vi "Post-Uninstall Custom Action.vi"(10 "Variant":variant) -> (0 "error out":errorcluster)   [LabVIEW 2024]
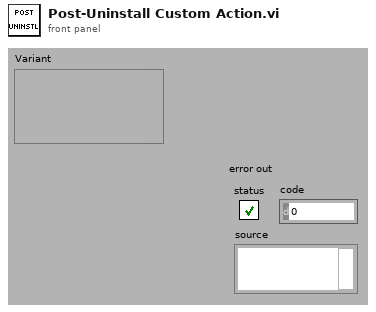
[diagram p1: front panel]
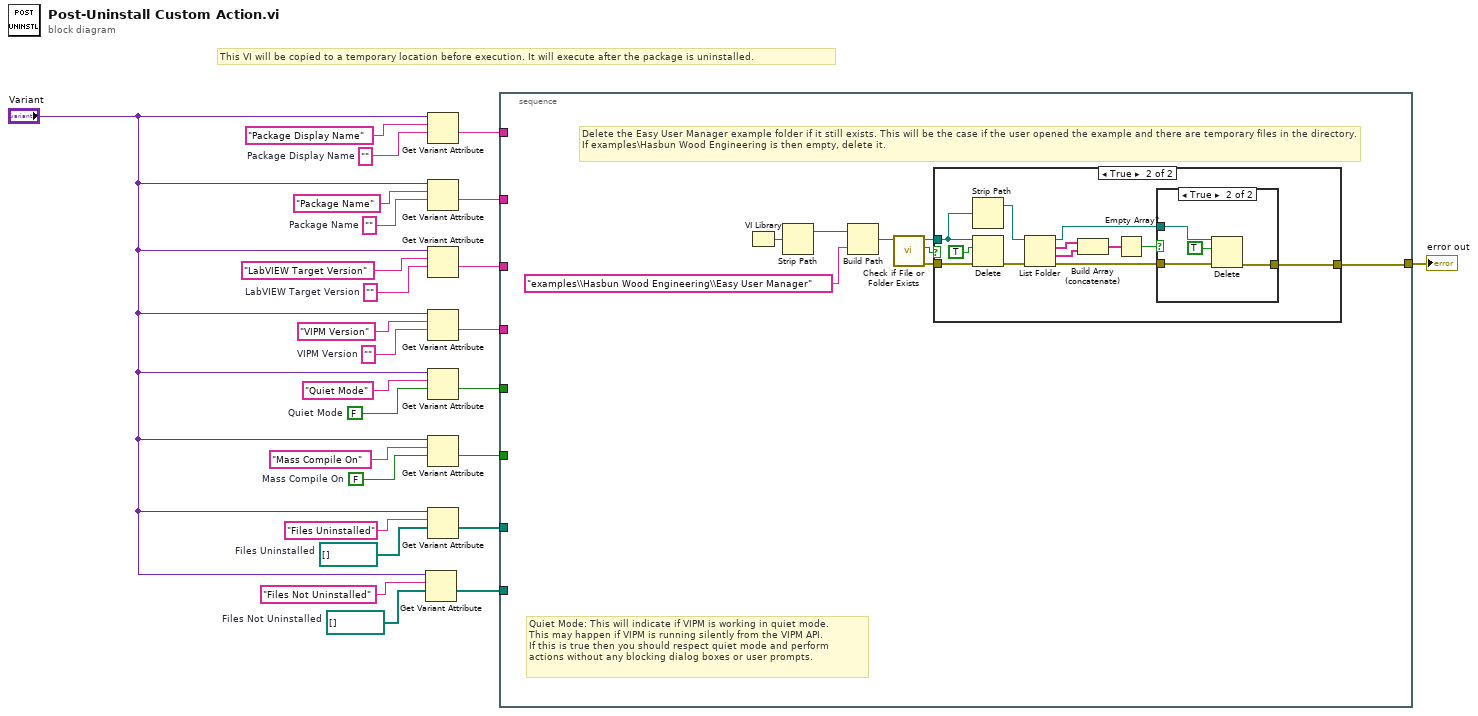
[diagram p0: block diagram]
diagram:
  w2 = path[] []  # Files Not Uninstalled
  w3 = path[] []  # Files Uninstalled
  w9 = FALSE  # Mass Compile On
  w10 = ""  # Package Display Name
  w17 = FALSE  # Quiet Mode
  w20 = ""  # VIPM Version
  w22 = ""  # LabVIEW Target Version
  w24 = ""  # Package Name
  # "This VI will be copied to a temporary location before execution. It will execute after the package is uninstalled."
  n1 = Get Variant Attribute(Variant="Variant", name="Files Not Uninstalled", default value (empty Variant)=w2) -> (value=w7:path[])  [unwired: 1 in, 3 out]
  n2 = Get Variant Attribute(Variant="Variant", name="Package Display Name", default value (empty Variant)=w10) -> (value=w16:string)  [unwired: 1 in, 3 out]
  n3 = Get Variant Attribute(Variant="Variant", name="Package Name", default value (empty Variant)=w24) -> (value=w15:string)  [unwired: 1 in, 3 out]
  n4 = Get Variant Attribute(Variant="Variant", name="LabVIEW Target Version", default value (empty Variant)=w22) -> (value=w14:string)  [unwired: 1 in, 3 out]
  n5 = Get Variant Attribute(Variant="Variant", name="VIPM Version", default value (empty Variant)=w20) -> (value=w13:string)  [unwired: 1 in, 3 out]
  n6 = Get Variant Attribute(Variant="Variant", name="Quiet Mode", default value (empty Variant)=w17) -> (value=w12:bool)  [unwired: 1 in, 3 out]
  n7 = Get Variant Attribute(Variant="Variant", name="Mass Compile On", default value (empty Variant)=w9) -> (value=w11:bool)  [unwired: 1 in, 3 out]
  n8 = Get Variant Attribute(Variant="Variant", name="Files Uninstalled", default value (empty Variant)=w3) -> (value=w6:path[])  [unwired: 1 in, 3 out]
  n9 = stacked-sequence {
    tunnel: w16 -> [_]
    tunnel: w15 -> [_]
    tunnel: w14 -> [_]
    tunnel: w13 -> [_]
    tunnel: w12 -> [_]
    tunnel: w11 -> [_]
    tunnel: w6 -> [_]
    tunnel: w7 -> [_]
    tunnel: [w27] -> w1
    frame #0 {
      # "Quiet Mode: This will indicate if VIPM is working in quiet mode.\nThis may happen if VIPM is running silently from the VIPM API.\nIf this is true then you should respect quiet mode and perform\nactions without any blocking dialog boxes or user prompts."
      # "Delete the Easy User Manager example folder if it still exists. This will be the case if the user opened the example and there are temporary files in the directory. If examples\\Hasbun Wood Engineering is then empty, delete it."
      n10 = VI Library() -> (path=w34:path)
      n11 = Strip Path(path=w34) -> (stripped path=w33:path)  [unwired: 1 out]
      n12 = Build Path(base path=w33, name or relative path="examples\\Hasbun Wood Engineering\\Easy User Manager") -> (appended path=w28:path)
      n13 = call <vilib>:"Check if File or Folder Exists.vi"("path"=w28) -> ("error out"=w29:errorcluster, "file or folder exists?"=w31:bool, "dup path"=w30:path)  [unwired: 8 in]
      n14 = case shown="True" w31 {
        tunnel: w30 -> [_ w36]
        tunnel: w29 -> [w35 w47]
        tunnel: [w35 w37] -> w27
        frame False {
        }
        frame True {
          n15 = Strip Path(path=w36) -> (stripped path=w45:path)  [unwired: 1 out]
          n16 = Delete(path (use dialog)=w36, entire hierarchy (F)=TRUE, error in=w47) -> (error out=w44:errorcluster)  [unwired: 2 in, 2 out]
          n17 = List Folder(path=w45, error in=w44) -> (path out=w43:path, filenames=w41:string[], folder names=w40:string[], error out=w42:errorcluster)  [unwired: 2 in]
          n18 = Build Array (concatenate)(w41, w40) -> (w39:string[])
          n19 = Empty Array?(array=w39) -> (empty?=w38:bool)
          n20 = case shown="True" w38 {
            tunnel: w43 -> [_ w51]
            tunnel: w42 -> [w48 w50]
            tunnel: [w48 w49] -> w37
            frame False {
            }
            frame True {
              n21 = Delete(path (use dialog)=w51, entire hierarchy (F)=TRUE, error in=w50) -> (error out=w49:errorcluster)  [unwired: 2 in, 2 out]
            }
          }
        }
      }
    }
  }
  "error out" <- w1
